vi "Clear_logs.vi"(6 "error in (no error)":errorcluster, 9 "VISA resource name":refnum<visa-resource-name>) -> (0 "error out":errorcluster, 3 "RESULT":bool)   [LabVIEW 2021]
uses:
  10054_Control Folder/Support/Relay_no.ctl
panel:
  out "read buffer":string
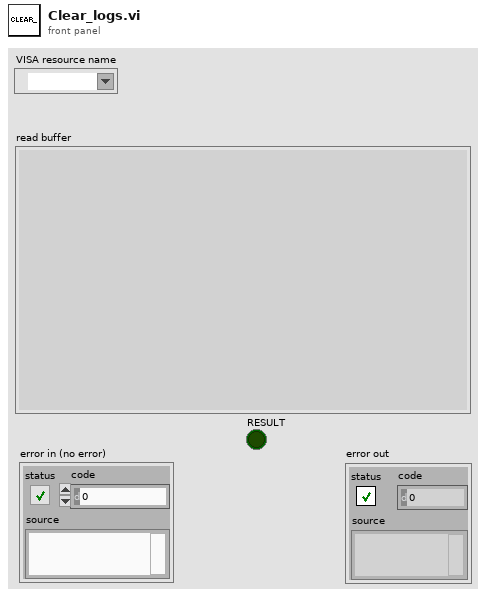
[diagram p1: front panel]
types:
  T1 = typedef "Relay_no.ctl" = enum16{"Init", "write&Read", "PCB Serial Write & Read", "PCB Write SSD & Password", "Read Wifi state", "Reset", "Close"}
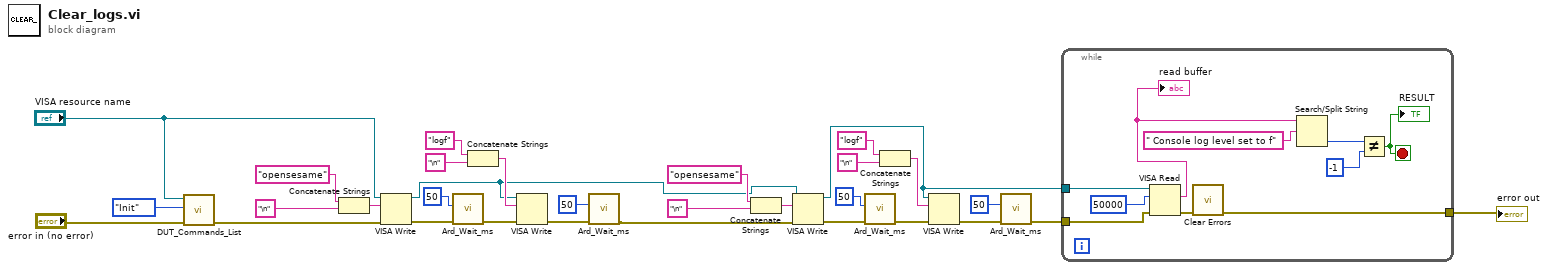
[diagram p0: block diagram]
diagram:
  n1 = call "DUT_Commands_List.vi"("error in"="error in (no error)", "Operation"=Relay_no."Init", "Resource In"="VISA resource name") -> ("error out"=w18:errorcluster)  [unwired: 6 in, 2 out]
  n2 = Concatenate Strings("opensesame" ("string"), "\n") -> (w27:string)
  n3 = VISA Write(VISA resource name="VISA resource name", write buffer=w27, error in (no error)=w18) -> (VISA resource name out=w2:refnum<visa-resource-name>, error out=w26:errorcluster)  [unwired: 1 out]
  n4 = call "Ard_Wait_ms.vi"("error in"=w26, "millisec"=u32 50) -> ("error in 2"=w30:errorcluster)  [unwired: 9 in]
  n5 = Concatenate Strings("logf" ("string"), "\n") -> (w28:string)
  n6 = VISA Write(VISA resource name=w2, write buffer=w28, error in (no error)=w30) -> (error out=w29:errorcluster)  [unwired: 2 out]
  n7 = call "Ard_Wait_ms.vi"("error in"=w29, "millisec"=u32 50) -> ("error in 2"=w4:errorcluster)  [unwired: 9 in]
  n8 = Concatenate Strings("opensesame" ("string"), "\n") -> (w8:string)
  n9 = VISA Write(VISA resource name=w2, write buffer=w8, error in (no error)=w4) -> (VISA resource name out=w1:refnum<visa-resource-name>, error out=w9:errorcluster)  [unwired: 1 out]
  n10 = call "Ard_Wait_ms.vi"("error in"=w9, "millisec"=u32 50) -> ("error in 2"=w5:errorcluster)  [unwired: 9 in]
  n11 = Concatenate Strings("logf" ("string"), "\n") -> (w7:string)
  n12 = VISA Write(VISA resource name=w1, write buffer=w7, error in (no error)=w5) -> (error out=w6:errorcluster)  [unwired: 2 out]
  n13 = call "Ard_Wait_ms.vi"("error in"=w6, "millisec"=u32 50) -> ("error in 2"=w3:errorcluster)  [unwired: 9 in]
  n14 = while {
    tunnel: w3 -> [w34]
    tunnel: w1 -> [w33]
    tunnel: [w32] -> w31
    stop <- w35 stop-if-true
    n15 = VISA Read(VISA resource name=w33, byte count=u32 50000, error in (no error)=w34) -> (read buffer=w36:string, error out=w40:errorcluster)  [unwired: 2 out]
    "read buffer" <- w36
    n16 = call <vilib>:"Clear Errors.vi"("error in (no error)"=w40) -> ("error out"=w32:errorcluster)  [unwired: 5 in, 1 out]
    n17 = Search/Split String(string=w36, search string/char (-)=" Console log level set to f") -> (offset of match=w38:i32)  [unwired: 1 in, 2 out]
    n18 = Not Equal?(x=w38, y=-1) -> (x != y?=w35:bool)
    "RESULT" <- w35
  }
  "error out" <- w31
